vi "Test-B.vi"() -> ()   [LabVIEW 2018]
uses:
  API.ctl
  678ff351-9fb4-42ed-b5b4-c7c4531d3cd8.vi
  <userlib>/_NEVSTOP/Communicable State Machine(CSM)/AdvanceAPI/CSM - Revert Arguments-Safe String.vi
  <userlib>/_NEVSTOP/Communicable State Machine(CSM)/_Shared/Trim Single-line Text.vi
  <userlib>/_NEVSTOP/Communicable State Machine(CSM)/AdvanceAPI/CSM - Make String Arguments Safe.vi
  <userlib>/_NEVSTOP/Communicable State Machine(CSM)/AdvanceAPI/CSM - Break Down Multiple States String.vi
  <userlib>/_NEVSTOP/Communicable State Machine(CSM)/AdvanceAPI/CSM - Compact Multiple States.vi
  <userlib>/_NEVSTOP/Communicable State Machine(CSM)/AdvanceAPI/CSM - Keywords.vi
  <userlib>/_NEVSTOP/Communicable State Machine(CSM)/addons/API-String-Arugments-Support/_Support/Data To API String Arguments.vi
  <userlib>/_NEVSTOP/Communicable State Machine(CSM)/_Polymophic/Build No-Reply Asynchronous Message with Arguments.vi
  <userlib>/_NEVSTOP/Communicable State Machine(CSM)/Communicable State Machine.lvlib
panel:
  out "Module Names":string[](array[string])
  out "连接的字符串":string
  in  "Timing Parameters":T1
  out "State History":string
  in  "UID)":string="Event CSM"
  in  "Send":bool
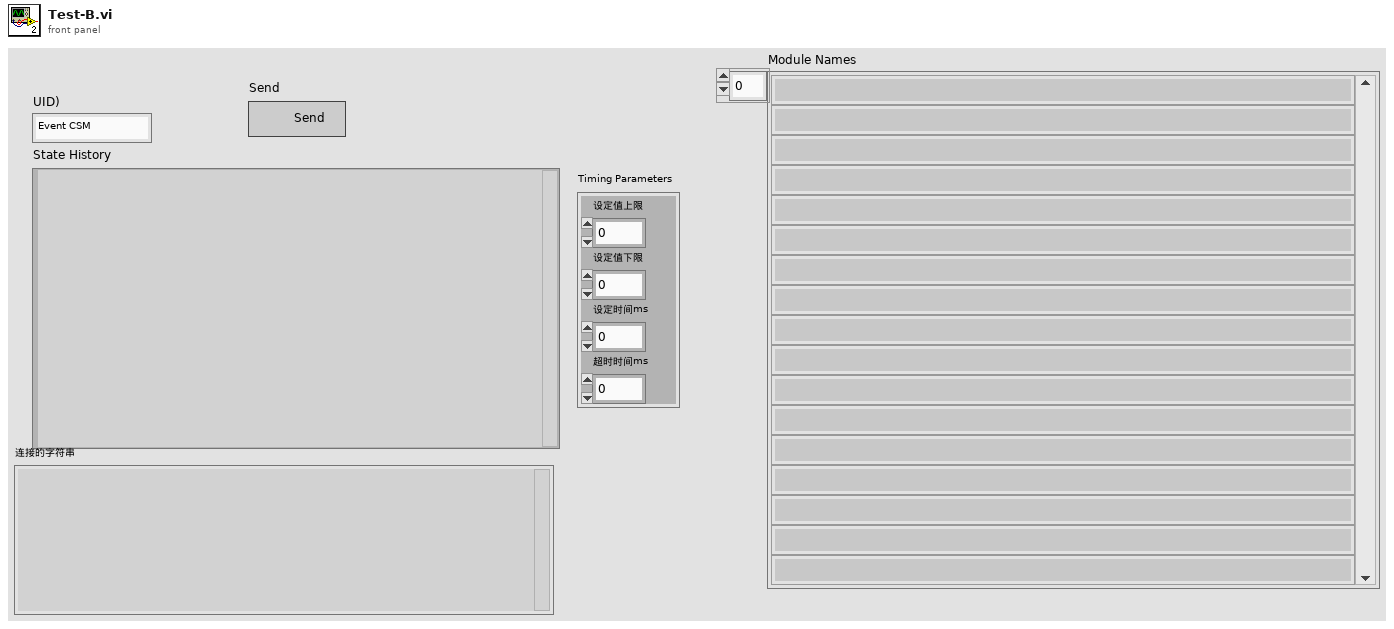
[diagram p1: front panel]
types:
  T1 = typedef "API.ctl" = cluster{"设定值上限":dbl, "设定值下限":dbl, "设定时间ms":u32, "超时时间ms":u32}
  T2 = enum32{"Invalid", "Standard", "Closed", "Hidden", "Minimized", "Maximized"}
  T3 = enum32{"invalid app kind", "Development System", "Run Time System", "Student Edition", "Embedded LabVIEW", "Evaluation", "Custom"}
  T4 = typedef "Communicable State Machine.lvlib/_CSM_Response Source Message.ctl" = cluster{"‘State":string, "’Arguments":string, "’Error":errorcluster}
  T5 = cluster{"Current VI Reference":refnum<vi>, "Close Panel on Exit?":bool}
  T6 = cluster{"Core":cluster{"Current VI Reference":refnum<vi>, "Close Panel on Exit?":bool}, "Your Boolean data":bool, "Your string data":string}
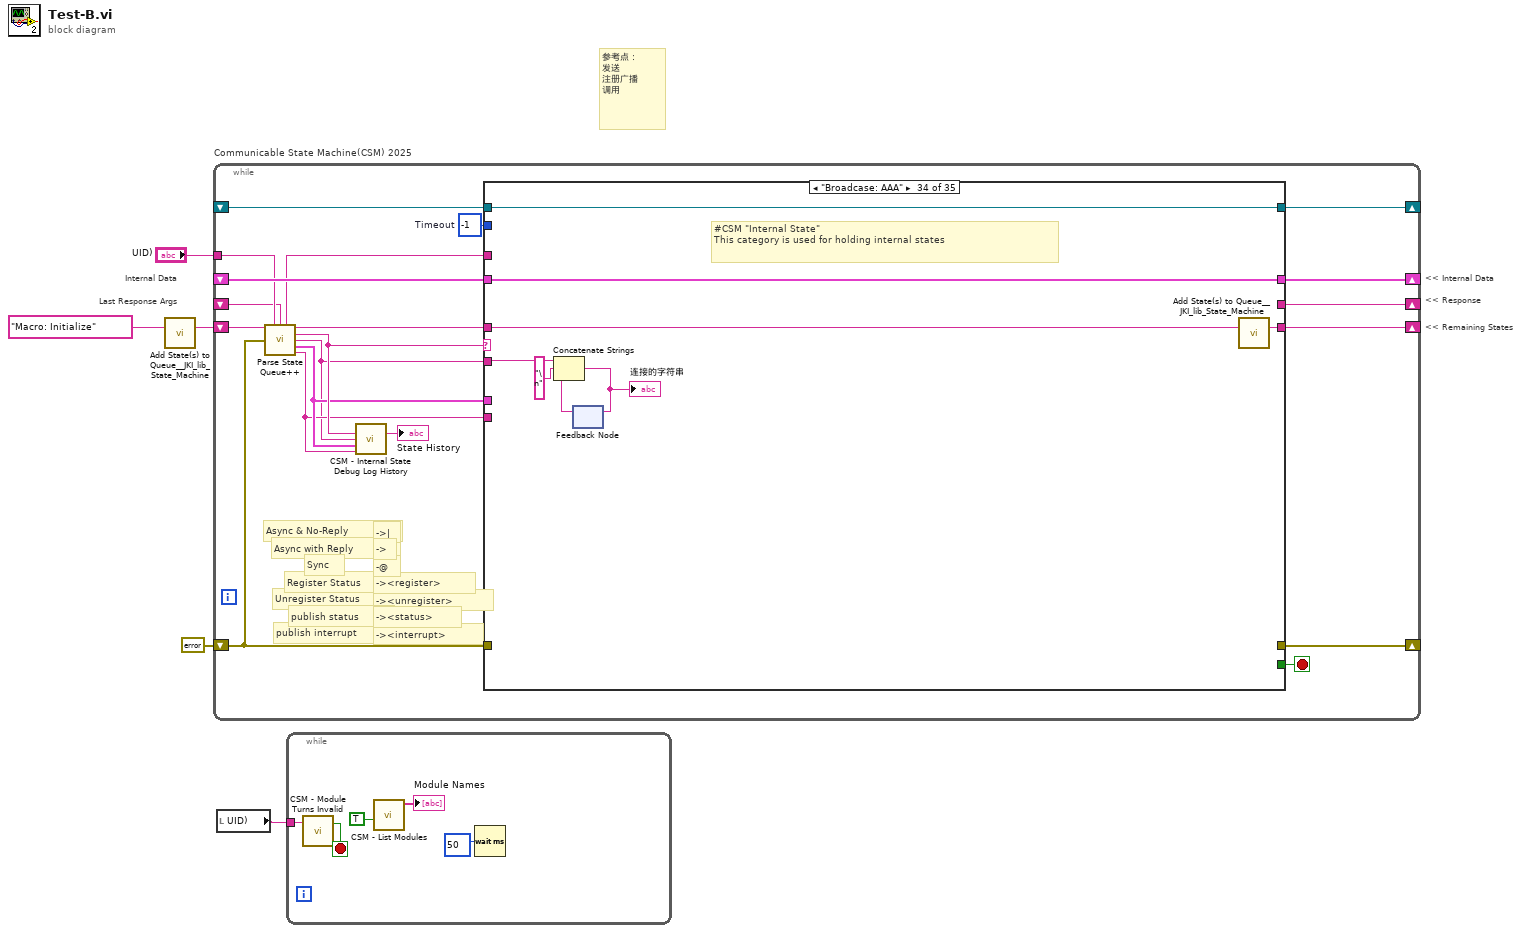
[diagram p0: block diagram]
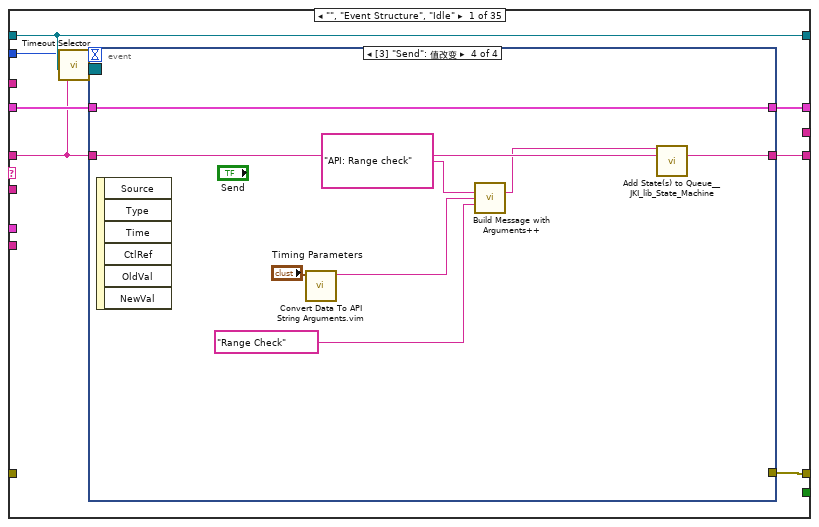
[diagram p2: hidden frame]
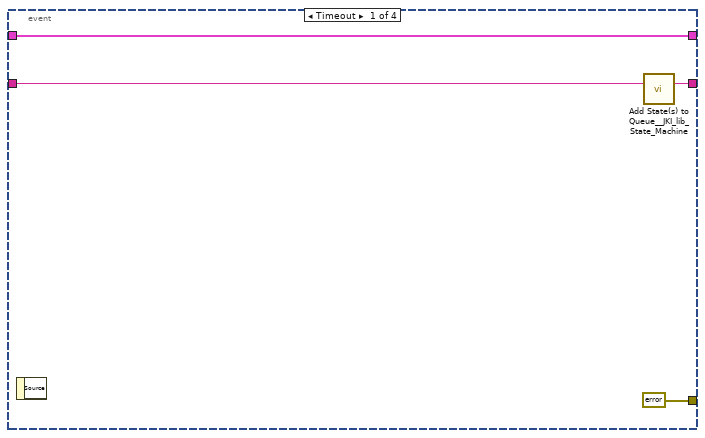
[diagram p3: hidden frame]
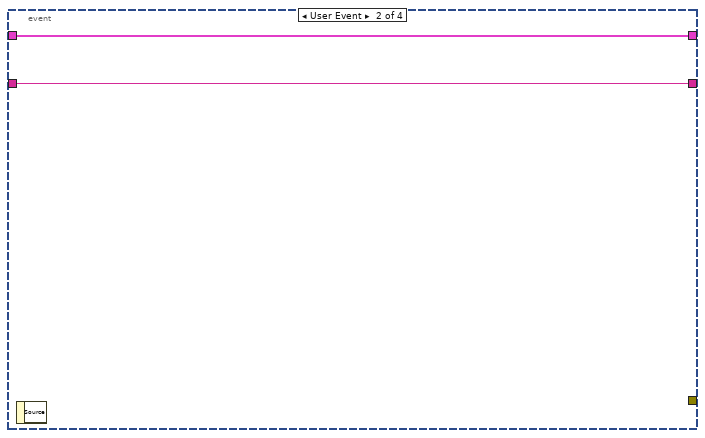
[diagram p4: hidden frame]
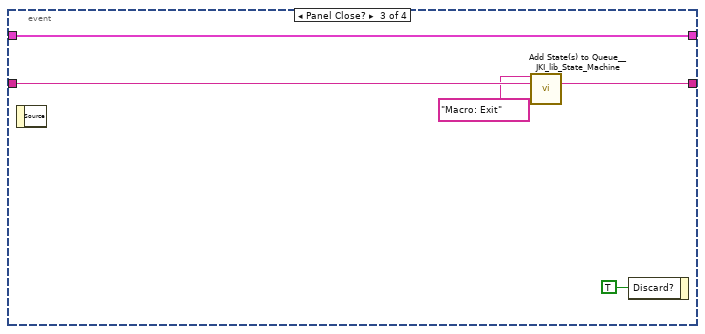
[diagram p5: hidden frame]
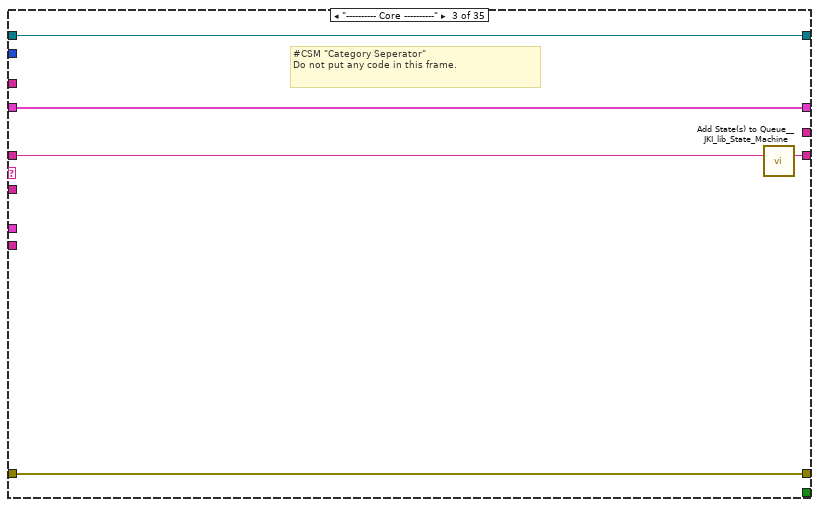
[diagram p7: hidden frame]
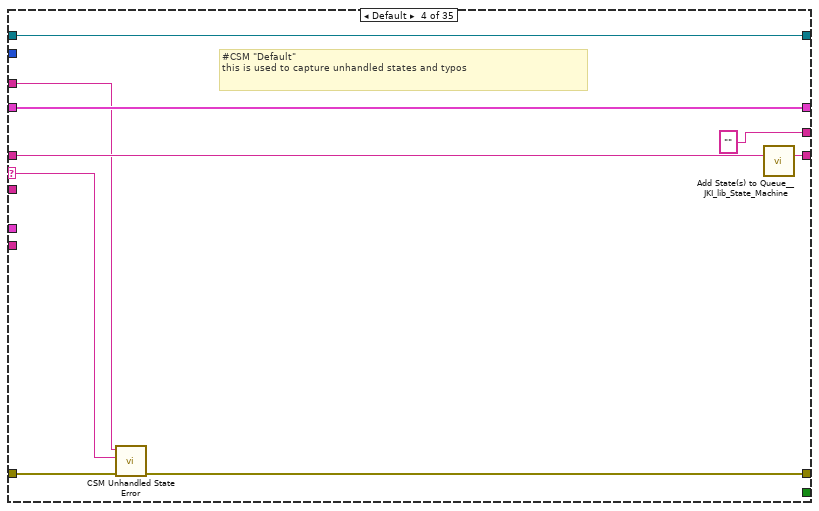
[diagram p8: hidden frame]
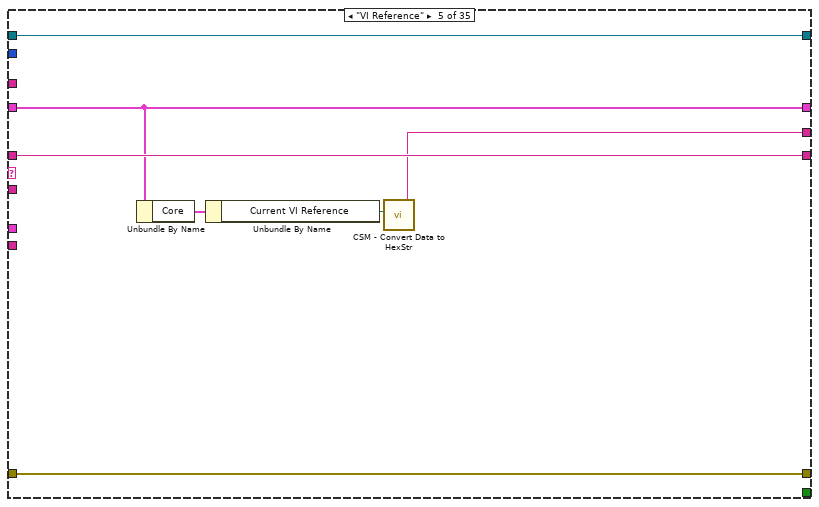
[diagram p9: hidden frame]
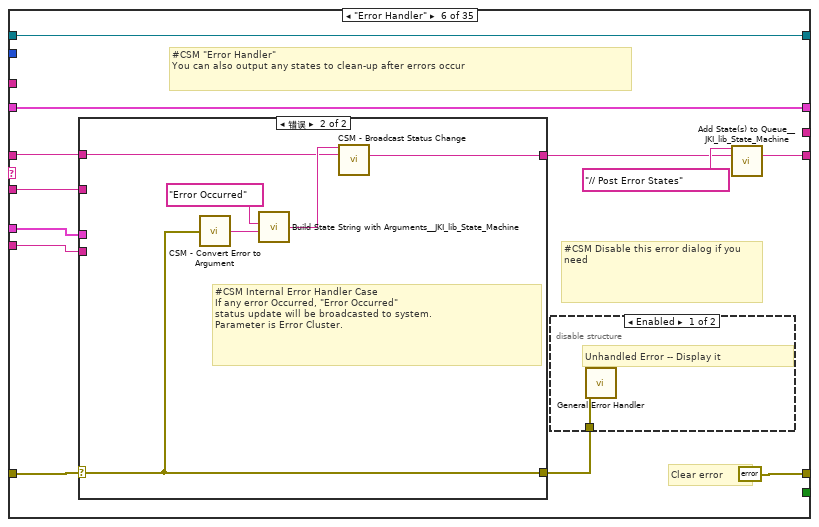
[diagram p10: hidden frame]
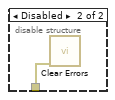
[diagram p11: hidden frame]
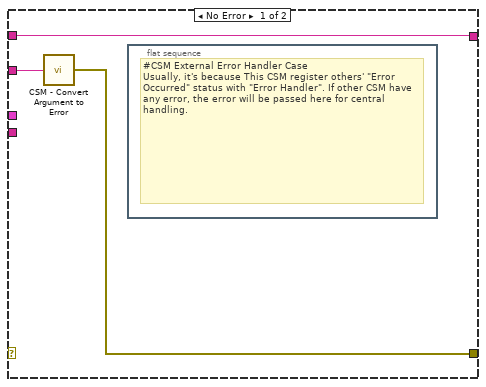
[diagram p12: hidden frame]
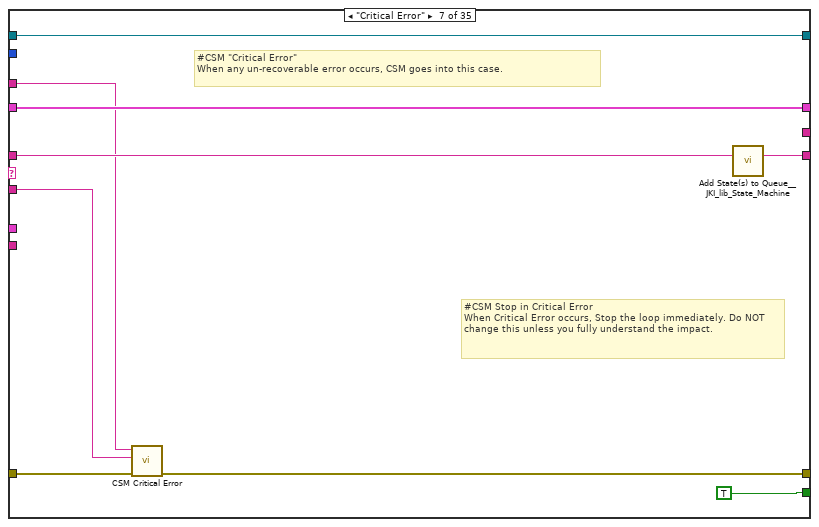
[diagram p13: hidden frame]
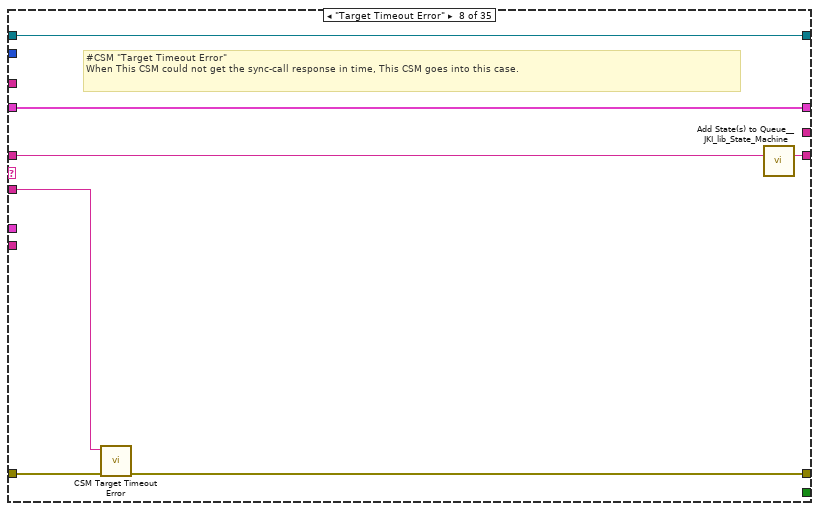
[diagram p14: hidden frame]
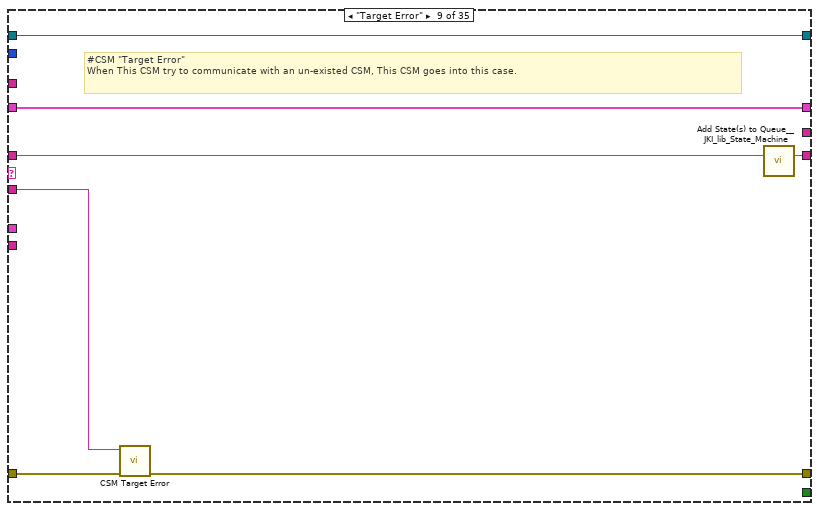
[diagram p15: hidden frame]
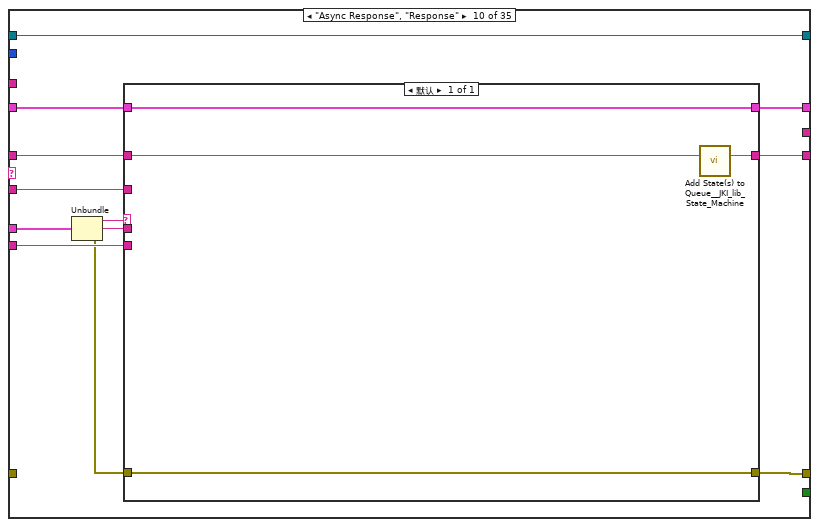
[diagram p16: hidden frame]
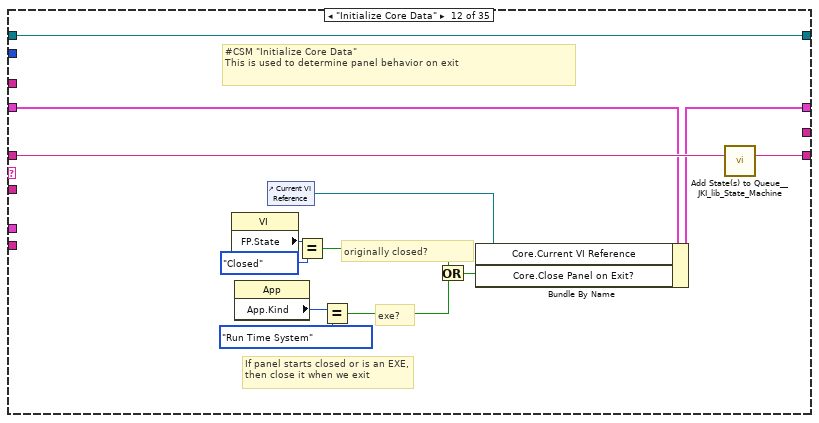
[diagram p18: hidden frame]
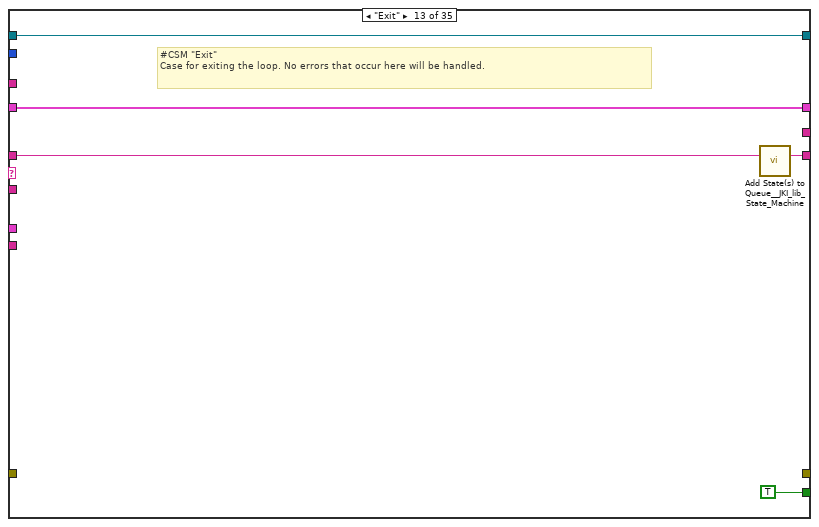
[diagram p19: hidden frame]
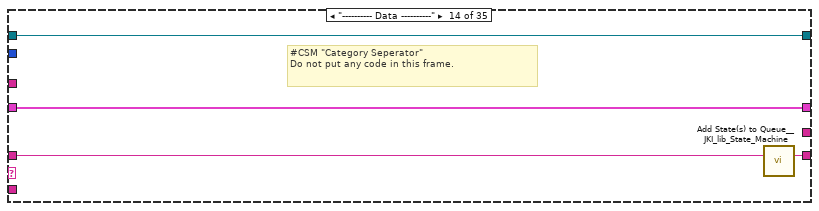
[diagram p20: hidden frame]
diagram:
  # "参考点：\n发送\n注册广播\n调用"
  # "Last Response Args"
  # "Internal Data"
  # "<< Internal Data"
  # "<< Response"
  # "<< Remaining States"
  n1 = call <vilib>:"Add State(s) to Queue__JKI_lib_State_Machine.vi"("State(s) in (\"\")"="Macro: Initialize" ("Init State(\"Macro: Initialize\")")) -> ("States Out"=w2:string)  [unwired: 14 in]
  n2 = while "Communicable State Machine(CSM) 2025" {
    shift-right: [w20] -> _
    shift-left: _ -> [w19]
    shift-right: [w23] -> _
    shift-left: errorcluster {"status"=FALSE, "code"=0, "source"=""} ("error out") -> [w17]
    shift-right: [w22] -> _
    shift-left: w2 -> [w24]
    tunnel: "UID)" -> [w13]
    shift-right: [w16] -> _
    shift-left: _ -> [w8]
    shift-right: [w15] -> _
    shift-left: _ -> [w14]
    stop <- w21 stop-if-true
    w18 = -1  # Timeout
    # "-><interrupt>"
    # "-><status>"
    # "-><unregister>"
    # "-><register>"
    # "-@"
    # "->"
    # "->|"
    # "publish interrupt"
    # "publish status"
    # "Unregister Status"
    # "Register Status"
    # "Sync"
    # "Async with Reply"
    # "Async & No-Reply"
    n3 = call <userlib>:"Parse State Queue++.vi"("State Queue"=w24, "Name (\"\" to Use UUID)"=w13, "Response Arguments"=w8, "Previous Error"=w17) -> ("Name Used"=w9:string, "Remaining States"=w25:string, "Current State"=w12:string, "Arguments"=w7:string, "Additional Information"=w11:T4, "Source CSM"=w10:string)  [unwired: 6 in]
    n4 = call <userlib>:"CSM - Internal State Debug Log History.vi"("State"=w12, "Arguments (\"\")"=w7, ">> Response Source Message >>"=w11, "Source (\"\")"=w10) -> ("Debug Log"=→"State History":string)  [unwired: 11 in]
    n5 = case shown="\"Broadcase: AAA\"" w12 {
      selector: w12 -> [_ _ _ w63 _ _ _ _ _ _ _ _ _ _ _ _ _ _ _ _ _ _ _ _ _ _ _ _ _ _ _ _ _ _ _]
      tunnel: w25 -> [w26 w55 w60 w69 w75 w81 w107 w115 w122 w132 w141 w154 w159 w163 w170 w176 w180 w187 w191 w195 w200 w221 w231 w236 w242 w253 w317 w322 w334 w337 w341 w344 w348 w356 w360]
      tunnel: w7 -> [_ _ _ _ _ w79 w103 w110 w118 w126 _ _ _ _ _ _ _ _ _ _ _ _ _ _ w238 w248 _ _ _ _ _ _ _ w352 _]
      tunnel: w19 -> [w32 w54 w57 w67 w74 w87 w108 w113 w120 w130 w140 w148 w157 w161 _ w172 w178 w186 w190 w193 w198 w219 w229 w234 w240 w250 w315 w320 w332 w336 w340 w343 w346 w354 w358]
      tunnel: [w31 _ w58 w61 w76 errorcluster {"status"=FALSE, "code"=0, "source"=""} ("error out") w100 w109 w116 w129 _ _ _ _ _ w173 _ w181 w189 _ _ _ _ _ w239 w251 _ _ _ _ _ _ _ _ _] -> w23
      tunnel: w17 -> [_ _ w58 w62 w76 w85 w101 w111 w117 _ _ _ _ _ _ _ _ _ _ _ _ _ _ _ _ _ _ _ _ _ _ _ _ _ _]
      tunnel: [w33 w55 w59 w68 w75 w83 w106 w114 w121 w133 w141 w153 w158 w162 w169 w175 w179 w187 w191 w194 w199 w220 w230 w235 w241 w252 w316 w321 w333 w337 w341 w344 w347 w355 w359] -> w22
      tunnel: [_ _ _ _ _ _ TRUE _ _ _ _ _ TRUE _ _ _ _ _ _ _ _ _ _ _ _ _ _ _ _ _ _ _ _ _ _] -> w21
      tunnel: [w30 w54 w57 w67 w74 w87 w108 w113 w120 w131 w140 w152 w157 w161 w168 w172 w178 w186 w190 w193 w198 w219 w229 w234 w240 w250 w315 w320 w332 w336 w340 w343 w346 w354 w358] -> w20
      tunnel: w18 -> [w28 _ _ _ _ _ _ _ _ _ _ _ _ _ _ _ _ _ _ _ _ _ _ _ _ _ _ _ _ _ _ _ _ _ _]
      tunnel: w10 -> [_ _ _ _ _ w78 _ _ _ w127 _ _ _ _ _ _ _ _ _ _ _ _ _ _ _ _ _ _ _ _ _ _ _ _ _]
      tunnel: w11 -> [_ _ _ _ _ w77 _ _ _ w128 _ _ _ _ _ _ _ _ _ _ _ _ _ _ _ _ _ _ _ _ _ _ _ _ _]
      tunnel: [_ _ _ "" w70 _ _ _ _ _ _ _ _ _ _ _ _ _ _ _ _ _ _ _ _ _ _ _ _ _ "API1 Response" _ _ _ _] -> w16
      tunnel: [w29 w53 w56 w65 w73 w86 w104 w112 w119 w134 w139 w142 w155 w160 w164 w171 w177 w185 w188 w192 w197 w218 w228 w233 w237 w247 w314 w318 w325 w335 w339 w342 w345 w353 w357] -> w15
      tunnel: w14 -> [w29 w53 w56 w65 w73 w86 w104 w112 w119 w134 w139 w142 w155 w160 w164 w171 w177 _ w188 w192 w197 w218 w228 w233 w237 w247 w314 w318 w325 w335 w339 w342 w345 w353 w357]
      tunnel: w9 -> [_ _ _ w64 _ _ w102 _ _ _ _ _ _ _ _ _ _ w184 _ _ _ _ _ _ _ _ _ _ _ _ _ _ _ _ _]
      frame "", "Event Structure", "Idle" {
        n6 = call <userlib>:"Timeout Selector.vi"("Remaining States"=w26, "Timeout Expected"=w28) -> ("Timeout"=w27:i32)  [unwired: 5 in]
        n7 = event shown="[3] \"Send\": 值改变" {
          selector: w29 -> [_ _ _ _]
          dyn-events: _ -> [_ _ _ _]
          timeout: w27 -> [_ _ _ _]
          tunnel: w26 -> [w37 w38 w44 w50]
          tunnel: [w36 w38 w43 w51] -> w33
          tunnel: w32 -> [w35 w39 w42 w52]
          tunnel: [errorcluster {"status"=FALSE, "code"=0, "source"=""} ("error out") _ _ _] -> w31
          tunnel: [w35 w39 w42 w52] -> w30
          event Timeout {
            n8 = event-data() -> ()  [unwired: 1 in, 1 out]
            n9 = call <vilib>:"Add State(s) to Queue__JKI_lib_State_Machine.vi"("State(s) in (\"\")"=w37) -> ("States Out"=w36:string)  [unwired: 14 in]
          }
          event User Event {
            n10 = event-data() -> ()  [unwired: 1 in, 1 out]
          }
          event Panel Close? {
            n11 = event-data() -> ()  [unwired: 1 in, 1 out]
            n12 = call <vilib>:"Add State(s) to Queue__JKI_lib_State_Machine.vi"("State(s) in Front (\"\")"="Macro: Exit", "State(s) in (\"\")"=w44) -> ("States Out"=w43:string)  [unwired: 13 in]
            n13 = event-data("Discard?"=TRUE) -> ()  [unwired: 1 in, 1 out]
          }
          event "Send": Value Change {
            n14 = event-data() -> ()  [unwired: 1 in, 6 out]
            n15 = call "Convert Data To API String Arguments.vim"("Data"="Timing Parameters") -> ("API String"=w46:string)  [unwired: 7 in, 1 out]
            n16 = call-poly <userlib>:"Build Message with Arguments++.vi"("State With Arguments"="API: Range check", "Arguments (\"\")"=w46, "Target Module (\"\")"="Range Check" ("Target Module (\"\")")) -> ("CSM Message String"=w48:string)  [unwired: 12 in]
            n17 = call <vilib>:"Add State(s) to Queue__JKI_lib_State_Machine.vi"("State(s) in Front (\"\")"=w48, "State(s) in (\"\")"=w50) -> ("States Out"=w51:string)  [unwired: 13 in]
          }
        }
      }
      frame "CSM Documentation" {
      }
      frame "---------- Core ----------" {
        # "#CSM \"Category Seperator\"\nDo not put any code in this frame."
        n18 = call <vilib>:"Add State(s) to Queue__JKI_lib_State_Machine.vi"("State(s) in (\"\")"=w60) -> ("States Out"=w59:string)  [unwired: 14 in]
      }
      frame Default {
        # "#CSM \"Default\"\nthis is used to capture unhandled states and typos"
        n19 = call <userlib>:"CSM Unhandled State Error.vi"("error in (no error)"=w62, "Undefined State"=w63, "CSM Name"=w64) -> ("error out"=w61:errorcluster)  [unwired: 8 in]
        n20 = call <vilib>:"Add State(s) to Queue__JKI_lib_State_Machine.vi"("State(s) in (\"\")"=w69) -> ("States Out"=w68:string)  [unwired: 14 in]
      }
      frame "VI Reference" {
        n21 = Unbundle By Name(w74) -> ("Core"=w72:T5)
        n22 = Unbundle By Name(w72) -> ("Current VI Reference"=w71:refnum<vi>)
        n23 = call <userlib>:"CSM - Convert Data to HexStr.vi"("Variant"=w71) -> ("HEX String (0-9,A-F)"=w70:string)  [unwired: 8 in]
      }
      frame "Error Handler" {
        # "#CSM Disable this error dialog if you need"
        # "#CSM \"Error Handler\"\nYou can also output any states to clean-up after errors occur"
        # "Clear error"
        n24 = case shown="错误" w85 {
          selector: w85 -> [_ w94]
          tunnel: [w92 w96] -> w82
          tunnel: w81 -> [w92 w95]
          tunnel: [w91 w94] -> w80
          tunnel: w79 -> [w93 _]
          tunnel: w78 -> [_ _]
          tunnel: w77 -> [_ _]
          frame No Error {
            n25 = call <userlib>:"CSM - Convert Argument to Error.vi"("Argument"=w93) -> ("Error"=w91:errorcluster)  [unwired: 4 in]
            n26 = flat-sequence {
              frame #0 {
                # "#CSM External Error Handler Case\nUsually, it's because This CSM register others' \"Error Occurred\" status with \"Error Handler\". If other CSM have any error, the error will be passed here for central handling."
              }
            }
          }
          frame Error {
            # "#CSM Internal Error Handler Case \nIf any error Occurred, \"Error Occurred\" \nstatus update will be broadcasted to system.\nParameter is Error Cluster."
            n27 = call <userlib>:"CSM - Convert Error to Argument.vi"("Error"=w94) -> ("Argument"=w98:string)  [unwired: 4 in]
            n28 = call <vilib>:"Build State String with Arguments__JKI_lib_State_Machine.vi"("Arguments (\"\")"=w98, "State"="Error Occurred" ("Status with Arguments")) -> ("State with Arguments"=w97:string)  [unwired: 4 in]
            n29 = call <userlib>:"CSM - Broadcast Status Change.vi"("Status With Arguments"=w97, "State Queue"=w95) -> ("Remaining States"=w96:string)  [unwired: 13 in]
          }
        }
        n30 = disable-structure shown="Enabled" {
          disable-tunnel: w80 -> [w89 w90]
          frame Enabled {
            # "Unhandled Error -- Display it"
            n31 = call <vilib>:"General Error Handler.vi"("error in (no error)"=w89) -> ()  [unwired: 10 in, 5 out]
          }
          frame Disabled {
            n32 = call <vilib>:"Clear Errors.vi"("error in (no error)"=w90) -> ()  [unwired: 5 in, 2 out]
          }
        }
        n33 = call <vilib>:"Add State(s) to Queue__JKI_lib_State_Machine.vi"("State(s) in Front (\"\")"="// Post Error States", "State(s) in (\"\")"=w82) -> ("States Out"=w83:string)  [unwired: 13 in]
      }
      frame "Critical Error" {
        # "#CSM \"Critical Error\"\nWhen any un-recoverable error occurs, CSM goes into this case."
        # "#CSM Stop in Critical Error\nWhen Critical Error occurs, Stop the loop immediately. Do NOT change this unless you fully understand the impact."
        n34 = call <userlib>:"CSM Critical Error.vi"("error in (no error)"=w101, "Arugments (As Reason)"=w103, "CSM Name"=w102) -> ("error out"=w100:errorcluster)  [unwired: 8 in]
        n35 = call <vilib>:"Add State(s) to Queue__JKI_lib_State_Machine.vi"("State(s) in (\"\")"=w107) -> ("States Out"=w106:string)  [unwired: 14 in]
      }
      frame "Target Timeout Error" {
        # "#CSM \"Target Timeout Error\"\nWhen This CSM could not get the sync-call response in time, This CSM goes into this case."
        n36 = call <userlib>:"CSM Target Timeout Error.vi"("error in (no error)"=w111, "Arguments (As CSM Name)"=w110) -> ("error out"=w109:errorcluster)  [unwired: 9 in]
        n37 = call <vilib>:"Add State(s) to Queue__JKI_lib_State_Machine.vi"("State(s) in (\"\")"=w115) -> ("States Out"=w114:string)  [unwired: 14 in]
      }
      frame "Target Error" {
        # "#CSM \"Target Error\"\nWhen This CSM try to communicate with an un-existed CSM, This CSM goes into this case."
        n38 = call <userlib>:"CSM Target Error.vi"("error in (no error)"=w117, "Arguments (As CSM Name)"=w118) -> ("error out"=w116:errorcluster)  [unwired: 9 in]
        n39 = call <vilib>:"Add State(s) to Queue__JKI_lib_State_Machine.vi"("State(s) in (\"\")"=w122) -> ("States Out"=w121:string)  [unwired: 14 in]
      }
      frame "Async Response", "Response" {
        n40 = Unbundle(w128) -> ("‘State"=w125:string, "’Arguments"=w124:string, "’Error"=w123:errorcluster)
        n41 = case shown="默认" w125 {
          tunnel: [w135] -> w133
          tunnel: w132 -> [w136]
          tunnel: [w138] -> w131
          tunnel: w130 -> [w138]
          tunnel: [w137] -> w129
          tunnel: w123 -> [w137]
          tunnel: w127 -> [_]
          tunnel: w126 -> [_]
          tunnel: w124 -> [_]
          frame 默认 {
            n42 = call <vilib>:"Add State(s) to Queue__JKI_lib_State_Machine.vi"("State(s) in (\"\")"=w136) -> ("States Out"=w135:string)  [unwired: 14 in]
          }
        }
      }
      frame "Async Message Posted" {
        # "#CSM \"Async Message Posted\"\nAfter Async Message is posted (-> or ->| ), CSM goes to this state for post-action.\nYou can use Argument - State to tell which Async Message is called."
      }
      frame "Initialize Core Data" {
        # "#CSM \"Initialize Core Data\"\nThis is used to determine panel behavior on exit"
        # "originally closed?"
        # "exe?"
        # "If panel starts closed or is an EXE, then close it when we exit"
        n43 = property class="VI"() -> ("FP.State"=w145:T2)  [unwired: 2 in, 2 out]
        n44 = property class="App"() -> ("App.Kind"=w151:T3)  [unwired: 2 in, 2 out]
        n45 = control-ref of="Current VI Reference"() -> (w146:refnum<vi>)
        n46 = Equal?(x=w145, y=T2."Closed" ("Front Panel Window:State")) -> (x = y?=w143:bool)
        n47 = Equal?(x=w151, y=T3."Run Time System" ("Application:Kind")) -> (x = y?=w149:bool)
        n48 = Or(x=w143, y=w149) -> (x .or. y?=w147:bool)
        n49 = Bundle By Name(cluster=w148, "Core.Current VI Reference"=w146, "Core.Close Panel on Exit?"=w147) -> (w152:T6)
        n50 = call <vilib>:"Add State(s) to Queue__JKI_lib_State_Machine.vi"("State(s) in (\"\")"=w154) -> ("States Out"=w153:string)  [unwired: 14 in]
      }
      frame "Exit" {
        # "#CSM \"Exit\"\nCase for exiting the loop. No errors that occur here will be handled."
        n51 = call <vilib>:"Add State(s) to Queue__JKI_lib_State_Machine.vi"("State(s) in (\"\")"=w159) -> ("States Out"=w158:string)  [unwired: 14 in]
      }
      frame "---------- Data ----------" {
        # "#CSM \"Category Seperator\"\nDo not put any code in this frame."
        n52 = call <vilib>:"Add State(s) to Queue__JKI_lib_State_Machine.vi"("State(s) in (\"\")"=w163) -> ("States Out"=w162:string)  [unwired: 14 in]
      }
      frame "Data: Initialize" {
        w165 = T5 {"Current VI Reference"=refnum, "Close Panel on Exit?"=FALSE}  # Core
        w167 = TRUE  # Your Boolean data
        w166 = ""  # Your string data
        # "#CSM  do not delete - used by framework"
        # "#CSM Expand Bundle to add new data elements to shift register data."
        # "#CSM Add new data here."
        # "#CSM Data names and types of shift register data are defined by this bundle."
        # "#CSM \"Data: Initialize\"\nInitialize the shift-register data, here.\n(data names are defined by what you wire into the bundle function)"
        n53 = Bundle("Core"=w165, "Your Boolean data"=w167, "Your string data"=w166) -> (w168:T6)  [unwired: 1 in]
        n54 = call <vilib>:"Add State(s) to Queue__JKI_lib_State_Machine.vi"("State(s) in (\"\")"=w170) -> ("States Out"=w169:string)  [unwired: 14 in]
      }
      frame "Data: Cleanup" {
        # "#CSM \"Data: Cleanup\"\nCleanup any data and references, here.\n(this is called automatically, by the Macro: Exit)"
        n55 = Unbundle By Name(w172) -> ("Core.Current VI Reference"=w174:refnum<vi>)
        n56 = Close Reference(reference=w174) -> (error out=w173:errorcluster)  [unwired: 1 in]
        n57 = call <vilib>:"Add State(s) to Queue__JKI_lib_State_Machine.vi"("State(s) in (\"\")"=w176) -> ("States Out"=w175:string)  [unwired: 14 in]
      }
      frame "---------- Events ----------" {
        # "#CSM \"Category Seperator\"\nDo not put any code in this frame."
        n58 = call <vilib>:"Add State(s) to Queue__JKI_lib_State_Machine.vi"("State(s) in (\"\")"=w180) -> ("States Out"=w179:string)  [unwired: 14 in]
      }
      frame "Events: Register" {
        # "#CSM \"Events: Register\"\nRegister user event. New Message Event is registered to break CSM waiting in event structure by default."
        # "#CSM Register New Message Event\nRegister message event to break Waiting in Event structure."
        n59 = call <userlib>:"CSM - Get New State Notifier Event.vi"("Name (\"\" to Use UUID)"=w184) -> ("error out"=w182:errorcluster, "New State Notifier Event"=w183:refnum<user-event>)  [unwired: 9 in]
        n60 = register-events(error in=w182, w183) -> (reference out=w185:refnum<event-registration>, error out=w181:errorcluster)  [unwired: 1 in]
      }
      frame "Events: Unregister" {
        # "#CSM \"Events: Unregister\"\nUnregister user event."
        n61 = Unregister For Events(event registration refnum=w188) -> (error out=w189:errorcluster)  [unwired: 1 in]
      }
      frame "---------- User Initialize ----------" {
        # "#CSM \"Category Seperator\"\nDo not put any code in this frame."
        n62 = call <vilib>:"Add State(s) to Queue__JKI_lib_State_Machine.vi"("State(s) in (\"\")"=w195) -> ("States Out"=w194:string)  [unwired: 14 in]
      }
      frame "UI: Initialize calling Timer" {
        n63 = for {
          N: 1 -> [_]
          w203 = "Range Check#"  # Name ("" to Use UUID)
          n64 = vi-ref "Range-check-csm-works.vi"() -> (w205:refnum<vi>)
          n65 = property class="VI接口类型2"(reference=w205) -> (reference out=w209:refnum<vi>, error out=w207:errorcluster, "Path"=w206:path)  [unwired: 1 in]
          n66 = Open VI Reference(type specifier VI Refnum (for type only)=w209, vi path=w206, options=128, error in (no error)=w207) -> (vi reference=w208:refnum<vi>, error out=w204:errorcluster)  [unwired: 2 in]
          n67 = call-by-ref "Start Asynchronous Call"(reference=w208, error in=w204, "UUID"=w203) -> (reference out=w201:refnum<vi>, error out=w202:errorcluster)  [unwired: 11 in]
          n68 = Close Reference(reference=w201, error in (no error)=w202) -> ()  [unwired: 1 out]
        }
        n69 = call <vilib>:"Add State(s) to Queue__JKI_lib_State_Machine.vi"("State(s) in (\"\")"=w200) -> ("States Out"=w199:string)  [unwired: 14 in]
      }
      frame "UI: Register Broadcast" {
        # "#CSM \"Category Seperator\"\nDo not put any code in this frame."
        n70 = call <userlib>:"CSM - List Modules.vi"("With Nodes? (F)"=TRUE) -> ("Module Names"=w216:string[])  [unwired: 9 in, 1 out]
        n71 = for {
          tunnel: w216 -> [w222] mode=indexing
          tunnel: [w226] -> w217 mode=indexing if=w227
          tunnel: "Range Check Completd@%s>>Broadcase: AAA-><register>" ("格式字符串") -> [w225]
          n72 = Format Into String(format string=w225, w222) -> (resulting string=w226:string)  [unwired: 2 in, 1 out]
          n73 = Match Pattern(string=w222, regular expression="Range Check" ("正则表达式")) -> (offset past match=w223:i32)  [unwired: 1 in, 3 out]
          n74 = Greater Or Equal To 0?(x=w223) -> (x >= 0?=w227:bool)
        }
        n75 = Array To Spreadsheet String(delimiter (Tab)="\n" ("分隔符(Tab)"), array=w217, 3:"" ("格式字符串")) -> (spreadsheet string=w211:string)
        n76 = call <vilib>:"Add State(s) to Queue__JKI_lib_State_Machine.vi"("State(s) in (\"\")"=w221, "State(s) at Back (\"\")"=w211) -> ("States Out"=w220:string)  [unwired: 13 in]
      }
      frame "---------- UI ----------" {
        # "#CSM \"Category Seperator\"\nDo not put any code in this frame."
        n77 = call <vilib>:"Add State(s) to Queue__JKI_lib_State_Machine.vi"("State(s) in (\"\")"=w231) -> ("States Out"=w230:string)  [unwired: 14 in]
      }
      frame "UI: Initialize" {
        # "#CSM \"UI: Initialize\"\nInitialize the User Interface, here.\n(this is called automatically, by the Macro: Init)"
        n78 = local write "连接的字符串"("" ("连接的字符串")) -> ()
        n79 = call <vilib>:"Add State(s) to Queue__JKI_lib_State_Machine.vi"("State(s) in (\"\")"=w236) -> ("States Out"=w235:string)  [unwired: 14 in]
      }
      frame "UI: Cursor Set" {
        # "Argument"
        # "#CSM \"UI: Cursor Set\"\nSet and Unset Cursor Busy.\n(Usage: \"UI: Cursor Set >> Busy|Idle\")"
        n80 = disable-structure shown="TARGET_TYPE!=Windows" {
          disable-tunnel: [w244 _] -> w239
          disable-tunnel: w238 -> [w243 _]
          frame condition #0 (active) {
            n81 = case shown="\"Idle\", 默认" w243 {
              tunnel: [w245 w246] -> w244
              frame "Idle", Default {
                n82 = call <vilib>:"Unset Busy.vi"() -> ("error out"=w245:errorcluster)  [unwired: 11 in]
              }
              frame "Busy" {
                n83 = call <vilib>:"Set Busy.vi"() -> ("error out"=w246:errorcluster)  [unwired: 10 in, 1 out]
              }
            }
          }
          frame condition #1 {
          }
        }
        n84 = call <vilib>:"Add State(s) to Queue__JKI_lib_State_Machine.vi"("State(s) in (\"\")"=w242) -> ("States Out"=w241:string)  [unwired: 14 in]
      }
      frame "UI: Front Panel State" {
        # "Argument"
        # "#CSM \"UI: Front Panel State\"\nSet Front Panel Open or Closed\n(Usage: \"UI: Front Panel State >> Open|Close\")"
        n85 = Unbundle By Name(w250) -> ("Core.Current VI Reference"=w249:refnum<vi>)
        n86 = case shown="\"Minimize\", \"Minimized\"" w248 {
          tunnel: [w260 w273 w284 w296 w308] -> w251
          tunnel: w249 -> [w259 w271 w283 w295 w307]
          frame "Open", "Standard", Default {
            w254 = T2."Standard" ("State")
            n87 = property class="VI"(reference=w259) -> (reference out=w257:refnum<vi>, error out=w258:errorcluster, "FP.State"=w256:T2)  [unwired: 1 in]
            n88 = Not Equal?(x=w256, y=w254) -> (x != y?=w255:bool)
            n89 = case shown="真" w255 {
              tunnel: [w264 w266] -> w260
              tunnel: w258 -> [w263 w266]
              tunnel: w257 -> [w262 _]
              tunnel: w254 -> [w261 _]
              frame True {
                n90 = invoke class="VI" method="FP.Open"(reference=w262, error in=w263, "Activate"=TRUE, "State"=w261) -> (error out=w264:errorcluster)  [unwired: 1 in, 4 out]
              }
              frame False {
              }
            }
          }
          frame "Close", "Closed" {
            n91 = property class="VI"(reference=w271) -> (reference out=w270:refnum<vi>, error out=w272:errorcluster, "FP.State"=w268:T2)  [unwired: 1 in]
            n92 = Not Equal?(x=w268, y=T2."Closed" ("Front Panel Window:State")) -> (x != y?=w267:bool)
            n93 = case shown="真" w267 {
              tunnel: [w274 w277] -> w273
              tunnel: w272 -> [w274 w276]
              tunnel: w270 -> [_ w275]
              frame False {
              }
              frame True {
                n94 = invoke class="VI" method="FP.Close"(reference=w275, error in=w276) -> (error out=w277:errorcluster)  [unwired: 1 in, 2 out]
              }
            }
          }
          frame "Hidden", "Hide" {
            w278 = T2."Hidden" ("State")
            n95 = property class="VI"(reference=w283) -> (reference out=w281:refnum<vi>, error out=w282:errorcluster, "FP.State"=w280:T2)  [unwired: 1 in]
            n96 = Not Equal?(x=w280, y=w278) -> (x != y?=w279:bool)
            n97 = case shown="真" w279 {
              tunnel: [w288 w289] -> w284
              tunnel: w282 -> [w287 w289]
              tunnel: w281 -> [w286 _]
              tunnel: w278 -> [w285 _]
              frame True {
                n98 = invoke class="VI" method="FP.Open"(reference=w286, error in=w287, "State"=w285) -> (error out=w288:errorcluster)  [unwired: 2 in, 4 out]
              }
              frame False {
              }
            }
          }
          frame "Minimize", "Minimized" {
            w290 = T2."Minimized" ("State")
            n99 = property class="VI"(reference=w295) -> (reference out=w293:refnum<vi>, error out=w294:errorcluster, "FP.State"=w292:T2)  [unwired: 1 in]
            n100 = Not Equal?(x=w292, y=w290) -> (x != y?=w291:bool)
            n101 = case shown="假" w291 {
              tunnel: [w300 w301] -> w296
              tunnel: w294 -> [w299 w301]
              tunnel: w293 -> [w298 _]
              tunnel: w290 -> [w297 _]
              frame True {
                n102 = invoke class="VI" method="FP.Open"(reference=w298, error in=w299, "State"=w297) -> (error out=w300:errorcluster)  [unwired: 2 in, 4 out]
              }
              frame False {
              }
            }
          }
          frame "Maximize", "Maximized" {
            w302 = T2."Maximized" ("State")
            n103 = property class="VI"(reference=w307) -> (reference out=w305:refnum<vi>, error out=w306:errorcluster, "FP.State"=w304:T2)  [unwired: 1 in]
            n104 = Not Equal?(x=w304, y=w302) -> (x != y?=w303:bool)
            n105 = case shown="真" w303 {
              tunnel: [w312 w313] -> w308
              tunnel: w306 -> [w311 w313]
              tunnel: w305 -> [w310 _]
              tunnel: w302 -> [w309 _]
              frame True {
                n106 = invoke class="VI" method="FP.Open"(reference=w310, error in=w311, "State"=w309) -> (error out=w312:errorcluster)  [unwired: 2 in, 4 out]
              }
              frame False {
              }
            }
          }
        }
        n107 = call <vilib>:"Add State(s) to Queue__JKI_lib_State_Machine.vi"("State(s) in (\"\")"=w253) -> ("States Out"=w252:string)  [unwired: 14 in]
      }
      frame "---------- Macro ----------" {
        # "#CSM \"Category Seperator\"\nDo not put any code in this frame."
        n108 = call <vilib>:"Add State(s) to Queue__JKI_lib_State_Machine.vi"("State(s) in (\"\")"=w317) -> ("States Out"=w316:string)  [unwired: 14 in]
      }
      frame "Macro: Initialize" {
        w319 = "Data: Initialize\nInitialize Core Data\nEvents: Register\nUI: Initialize\nUI: Front Panel State >> Open\nUI: Initialize calling Timer\nUI: Register Broadcast"  # Data: Initialize Initialize Core Data Events: Register UI: Initialize UI: Front Panel State >> Open UI: Initialize calling Timer UI: Register Broadcast
        # "#CSM \"Macro: Initialize\"\nInitialization Macro (This is called once, when the VI starts)"
        n109 = call <vilib>:"Add State(s) to Queue__JKI_lib_State_Machine.vi"("State(s) in Front (\"\")"=w319, "State(s) in (\"\")"=w322) -> ("States Out"=w321:string)  [unwired: 13 in]
      }
      frame "Macro: Exit" {
        # "#CSM \"Macro: Exit\"\nExit Macro (This is called once, when the VI exits)"
        n110 = Unbundle By Name(w332) -> ("Core.Close Panel on Exit?"=w331:bool)
        n111 = call <userlib>:"CSM - Build Exit Messages of CSMs.vi"("CSMs"=string[] ["Range Check"]) -> ("States"=w324:string)  [unwired: 14 in]
        n112 = Select(t="UI: Front Panel State >> Close", s=w331, f="") -> (s? t:f=w328:string)
        n113 = call <vilib>:"Add State(s) to Queue__JKI_lib_State_Machine.vi"("State(s) in Front (\"\")"=w324, "State(s) in (\"\")"=w328, "State(s) at Back (\"\")"="Data: Cleanup\nEvents: Unregister\nExit") -> ("States Out"=w326:string)  [unwired: 12 in]
        n114 = call <vilib>:"Add State(s) to Queue__JKI_lib_State_Machine.vi"("State(s) in Front (\"\")"=w326, "State(s) in (\"\")"=w334) -> ("States Out"=w333:string)  [unwired: 13 in]
      }
      frame "---------- API ----------" {
        # "#CSM \"Category Seperator\"\nDo not put any code in this frame."
      }
      frame "API: API1" {
        # "#CSM >> Source CSM >>\nIf you need to tell who triggered this state , use this string. If it's this case itself, this string is \"\"."
        # "#CSM >> Arguments >>\nDeal with the parameter if any"
        # "#CSM Response\nConnect this to return the response of your API"
        # "#CSM API Example\nCopy/Rename this case for your own API"
      }
      frame "API: API2" {
        # "#CSM API Example\nCopy/Rename this case for your own API"
      }
      frame "---------- Broadcast ----------" {
        # "#CSM \"Category Seperator\"\nDo not put any code in this frame."
        n115 = call <vilib>:"Add State(s) to Queue__JKI_lib_State_Machine.vi"("State(s) in (\"\")"=w348) -> ("States Out"=w347:string)  [unwired: 14 in]
      }
      frame "Broadcase: AAA" {
        # "#CSM \"Internal State\"\nThis category is used for holding internal states"
        n116 = feedback #1() -> (w349:string)  [unwired: 1 in]
        n117 = Concatenate Strings(w352, "\n" ("字符串"), w349) -> (w350:string)
        "连接的字符串" <- w350
        n118 = feedback-in #1(w350) -> ()
        n119 = call <vilib>:"Add State(s) to Queue__JKI_lib_State_Machine.vi"("State(s) in (\"\")"=w356) -> ("States Out"=w355:string)  [unwired: 14 in]
      }
      frame "Brosdcase: action2" {
        # "#CSM \"Internal State\"\nThis category is used for holding internal states"
        n120 = call <vilib>:"Add State(s) to Queue__JKI_lib_State_Machine.vi"("State(s) in (\"\")"=w360) -> ("States Out"=w359:string)  [unwired: 14 in]
      }
    }
  }
  n121 = local read "UID)"() -> (w1:string)
  n122 = while {
    tunnel: w1 -> [w364]
    stop <- w363 stop-if-true
    n123 = call <userlib>:"CSM - Module Turns Invalid.vi"("CSM Name"=w364) -> ("Turn Invalid (Exit)?"=w363:bool)  [unwired: 2 in]
    n124 = call <userlib>:"CSM - List Modules.vi"("With Nodes? (F)"=TRUE) -> ("Module Names"=→"Module Names":string[])  [unwired: 9 in, 1 out]
    n125 = Wait (ms)(milliseconds to wait=u32 50 ("等待时间（毫秒）")) -> ()  [unwired: 1 out]
  }
